vi "Init.vi"(8 "error in (no error)":errorcluster, 11 "Data in":refnum<class "CTI_Serial_Bus.lvclass">) -> (0 "error out":errorcluster, 3 "Data out":refnum<class "CTI_Serial_Bus.lvclass">)   [LabVIEW 2021, in "CTI_Serial_Bus.lvclass"]
doc: "Abstract Data Classes 2.1.1.12\nTim Streeter - TSA\nCopyright (c) 2024, TSAOmni-Bus 2.0.1.6\nTim - TSA\nCopyright (c) 2024, TSA"
uses:
  CTI_Serial_Bus.lvclass
  C:/TSA/CTI_Bus/Source/Parent/CTI_Bus.lvclass
  Parent/CTI_Bus.lvclass/CTI_Bus.ctl
  CTI_Serial_Bus.lvclass/CTI_Serial_Bus.ctl
  Parent/Properties/Write Session.vi
  Parent/Properties/Write Identity.vi
  Parent/Properties/Read Error Checking.vi
  Parent/Properties/Read VISA resource name.vi
  Parent/CTI_Bus.lvclass
  <vilib>/CTI/CTI Drivers/CTI/VisaComms/VisaComms.lvclass
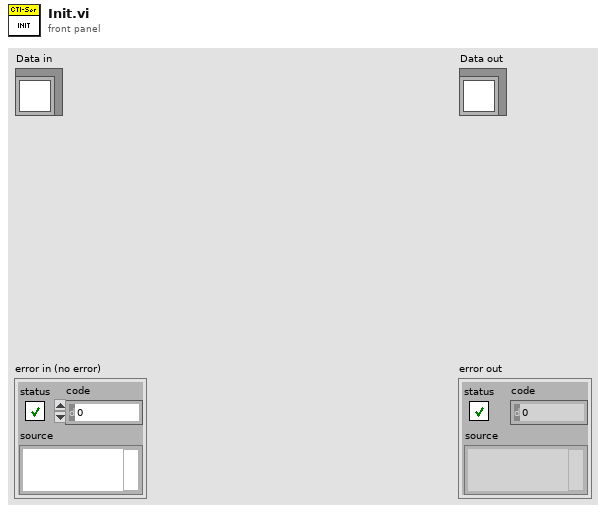
[diagram p1: front panel]
types:
  T1 = typedef "CTI.lvlib/Error Reporting.ctl" = enum16{"Minimal", "Moderate", "Full"}
  T2 = typedef "CTI.lvlib/Identity.ctl" = cluster{"Vendor":string, "Model":string, "Serial":string, "Version":string}
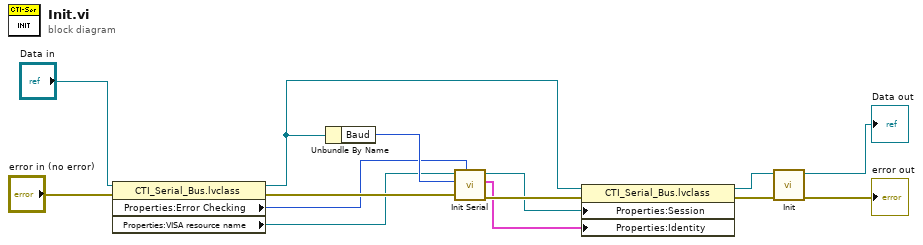
[diagram p0: block diagram]
diagram:
  n1 = property class="CTI_Serial_Bus.lvclass"(reference="Data in", error in="error in (no error)") -> (reference out=w8:refnum<class "CTI_Serial_Bus.lvclass">, error out=w7:errorcluster, "Properties:Error Checking"=w5:T1, "Properties:VISA resource name"=w6:refnum<visa-resource-name>)
  n2 = Unbundle By Name(w8) -> ("Baud"=w14:u32)
  n3 = call <vilib>:"Init Serial.vi"("Error Checking (Full)"=w5, "error in (no error)"=w7, "Baud (115200)"=w14, "VISA resource name in"=w6) -> ("error out"=w13:errorcluster, "Identity"=w11:T2, "Session"=w12:refnum<class "Session.lvclass">)  [unwired: 5 in]
  n4 = property class="CTI_Serial_Bus.lvclass"(reference=w8, error in=w13, "Properties:Session"=w12, "Properties:Identity"=w11) -> (reference out=w2:refnum<class "CTI_Serial_Bus.lvclass">, error out=w4:errorcluster)
  n5 = call-parent "Init.vi"("error in (no error)"=w4, "Data in"=w2) -> ("error out"=→"error out":errorcluster, "Data out"=→"Data out":refnum<class "CTI_Serial_Bus.lvclass">)  [unwired: 8 in]
